vi "Disconnect from Server.vi"(8 "error in (no error)":errorcluster, 11 "Client in":refnum<class "Client.lvclass">) -> (0 "error out":errorcluster, 1 "timed out":bool, 3 "Client out":refnum<class "Client.lvclass">)   [LabVIEW 2013, in "MQTT Client.lvlib" / "Client.lvclass"]
uses:
  Client.lvclass
  <vilib>/LabVIEW Open Source Project/MQTT Connection/MQTT_Base/Session/Session.lvclass/Session.ctl
  <vilib>/LabVIEW Open Source Project/MQTT Control Packets/Control Packets/DISCONNECT/DISCONNECT.lvclass
  Session.Client/Session.Client.lvclass
  <vilib>/LabVIEW Open Source Project/MQTT Connection/MQTT_Base/Session/Session.lvclass
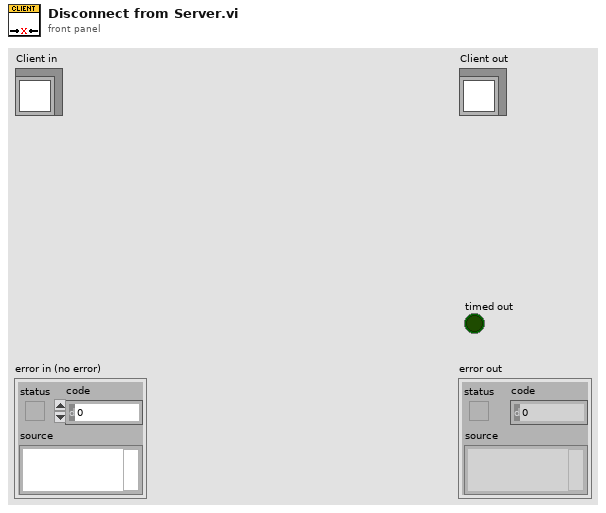
[diagram p1: front panel]
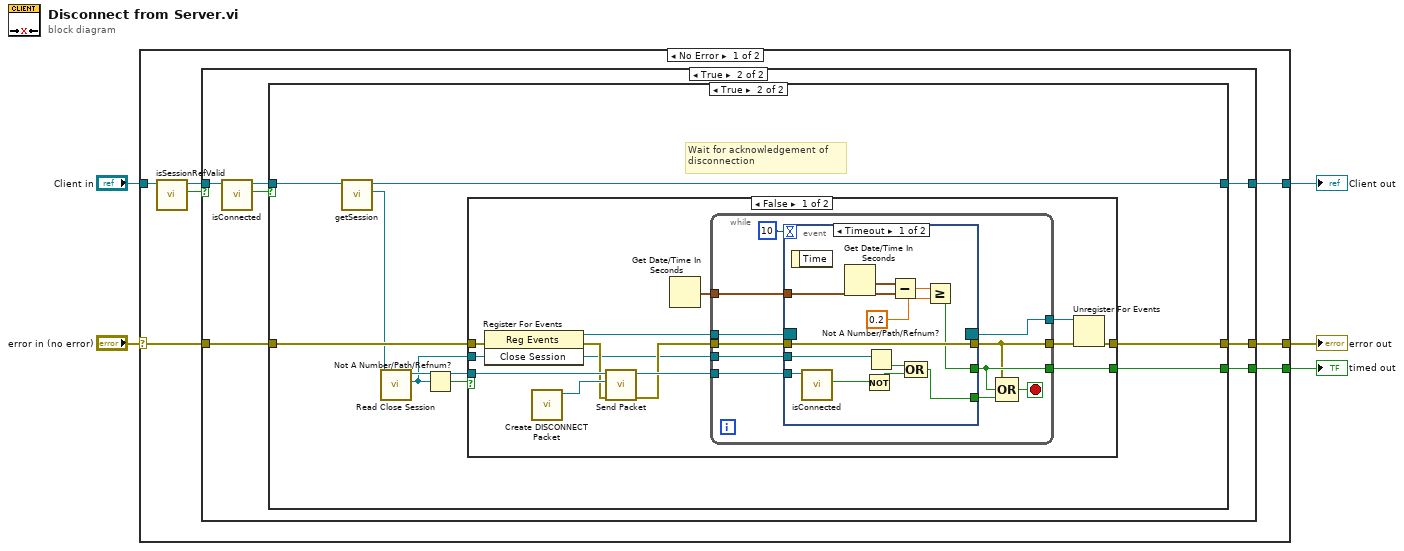
[diagram p0: block diagram]
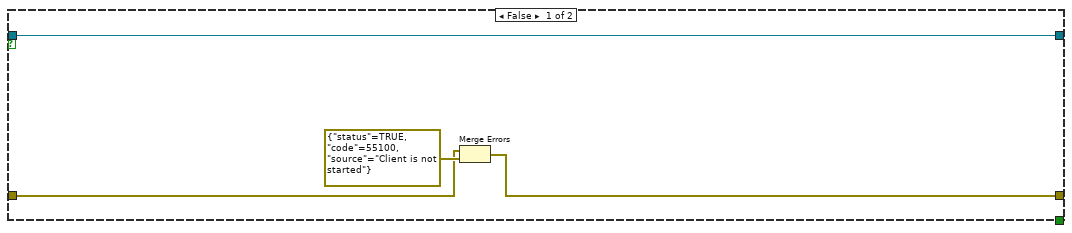
[diagram p2: hidden frame]
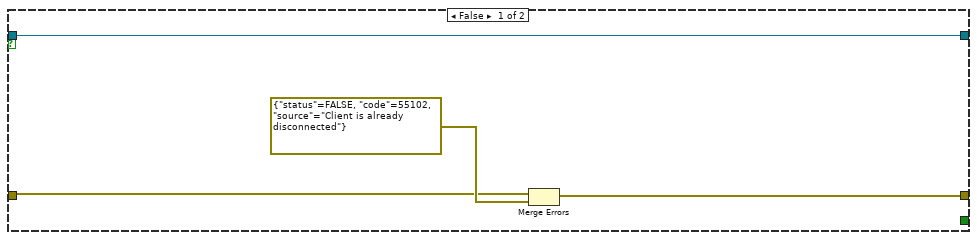
[diagram p3: hidden frame]
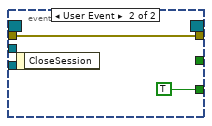
[diagram p4: hidden frame]
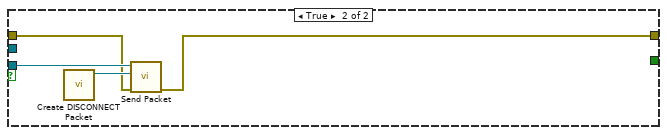
[diagram p5: hidden frame]
diagram:
  n1 = case shown="No Error" "error in (no error)" {
    selector: "error in (no error)" -> [w12 w80]
    tunnel: [w11 w80] -> w4
    tunnel: [w9 w79] -> w2
    tunnel: "Client in" -> [w8 w79]
    tunnel: [w10 _] -> w1
    frame No Error {
      n2 = call "isSessionRefValid.vi"("Client in"=w8) -> ("Session ref valid"=w7:bool, "Client out"=w6:refnum<class "Client.lvclass">)  [unwired: 9 in]
      n3 = case shown="True" w7 {
        tunnel: w12 -> [w14 w23]
        tunnel: [w13 w22] -> w11
        tunnel: [_ w21] -> w10
        tunnel: w6 -> [w16 w20]
        tunnel: [w16 w17] -> w9
        frame False {
          n4 = Merge Errors(w14, errorcluster {"status"=TRUE, "code"=55100, "source"="Client is not started"} ("error in")) -> (w13:errorcluster)
        }
        frame True {
          n5 = call <vilib>:"isConnected.vi"("Client in"=w20) -> ("connected"=w18:bool, "Client out"=w19:refnum<class "Client.lvclass">)  [unwired: 8 in, 1 out]
          n6 = case shown="True" w18 {
            tunnel: w23 -> [w25 w36]
            tunnel: [w24 w28] -> w22
            tunnel: [_ w35] -> w21
            tunnel: w19 -> [w27 w30]
            tunnel: [w27 w29] -> w17
            frame False {
              n7 = Merge Errors(w25, errorcluster {"status"=FALSE, "code"=55102, "source"="Client is already disconnected"} ("error in")) -> (w24:errorcluster)
            }
            frame True {
              # "Wait for acknowledgement of\ndisconnection"
              n8 = call "getSession.vi"("Client in"=w30) -> ("Session"=w31:refnum<class "Session.Client.lvclass">, "Client out"=w29:refnum<class "Client.lvclass">)  [unwired: 8 in, 1 out]
              n9 = call <vilib>:"Read Close Session.vi"("Session in"=w31) -> ("Close Session"=w32:refnum<user-event>, "Session out"=w33:refnum<class "Session.Client.lvclass">)  [unwired: 8 in, 1 out]
              n10 = Not A Number/Path/Refnum?(number/path/refnum=w32) -> (NaN/Path/Refnum?=w34:bool)
              n11 = case shown="False" w34 {
                tunnel: w36 -> [w49 w76]
                tunnel: [w48 w75] -> w28
                tunnel: [w47 _] -> w35
                tunnel: w33 -> [w41 w77]
                tunnel: w32 -> [w37 _]
                frame False {
                  n12 = register-events(error in=w49, w37) -> (reference out=w44:refnum<event-registration>, error out=w39:errorcluster)  [unwired: 1 in]
                  n13 = call <vilib>:"Create DISCONNECT Packet.vi"() -> ("DISCONNECT"=w42:refnum<class "DISCONNECT.lvclass">)  [unwired: 9 in, 2 out]
                  n14 = call "Send Packet.vi"("error in (no error)"=w39, "Packet"=w42, "Session"=w41) -> ("error out"=w38:errorcluster, "Session"=w40:refnum<class "Session.Client.lvclass">)  [unwired: 5 in, 2 out]
                  n15 = Get Date/Time In Seconds() -> (seconds since 1Jan1904=w43:timestamp)
                  n16 = while {
                    tunnel: [w54] -> w47
                    tunnel: [w60] -> w46
                    tunnel: [w53] -> w45
                    tunnel: w38 -> [w59]
                    tunnel: w44 -> [w58]
                    tunnel: w40 -> [w52]
                    tunnel: w37 -> [w51]
                    tunnel: w43 -> [w50]
                    stop <- w55 stop-if-true
                    n17 = event shown="[0] Timeout" {
                      selector: w58 -> [_ _]
                      dyn-events: [_ _] -> w60
                      timeout: 10 -> [_ _]
                      tunnel: [w72 w74] -> w53
                      tunnel: w59 -> [w72 w74]
                      tunnel: [w69 _] -> w54
                      tunnel: [w65 TRUE] -> w56
                      tunnel: w52 -> [w64 _]
                      tunnel: w51 -> [w68 _]
                      tunnel: w50 -> [w61 _]
                      event Timeout {
                        n18 = event-data() -> ()  [unwired: 1 in, 1 out]
                        n19 = call <vilib>:"isConnected.vi"("Session in"=w64) -> ("connected"=w63:bool)  [unwired: 8 in, 2 out]
                        n20 = Get Date/Time In Seconds() -> (seconds since 1Jan1904=w62:timestamp)
                        n21 = Not(x=w63) -> (.not. x?=w66:bool)
                        n22 = Not A Number/Path/Refnum?(number/path/refnum=w68) -> (NaN/Path/Refnum?=w67:bool)
                        n23 = Subtract(x=w62, y=w61) -> (x-y=w71:dbl)
                        n24 = Compound Arithmetic op=OR(w67, w66) -> (w65:bool)
                        n25 = Greater Or Equal?(x=w71, y=0.2) -> (x >= y?=w69:bool)
                      }
                      event User Event {
                        n26 = event-data() -> ()  [unwired: 1 in, 1 out]
                      }
                    }
                    n27 = Compound Arithmetic op=OR(w53, w54, w56) -> (w55:bool)
                  }
                  n28 = Unregister For Events(event registration refnum=w46, error in=w45) -> (error out=w48:errorcluster)
                }
                frame True {
                  n29 = call <vilib>:"Create DISCONNECT Packet.vi"() -> ("DISCONNECT"=w78:refnum<class "DISCONNECT.lvclass">)  [unwired: 9 in, 2 out]
                  n30 = call "Send Packet.vi"("error in (no error)"=w76, "Packet"=w78, "Session"=w77) -> ("error out"=w75:errorcluster)  [unwired: 5 in, 3 out]
                }
              }
            }
          }
        }
      }
    }
    frame Error {
    }
  }
  "error out" <- w4
  "Client out" <- w2
  "timed out" <- w1
